vi "Test Instrument Remote API.vi"   [LabVIEW 2019]
uses:
  <vilib>/JKI/JKI SMO/SMO/Typedefs/SMOState --Enum.ctl
  c5a0c80c-7090-426d-a2a1-7f80a9253fe7.vi
  c5a0c80c-7090-426d-a2a1-7f80a9253fe7.vi/3f0cefdb-5cc5-4526-b0b8-38505ee8bd1c.vi
  c5a0c80c-7090-426d-a2a1-7f80a9253fe7.vi/3f0cefdb-5cc5-4526-b0b8-38505ee8bd1c.vi/fd19d2b7-c57e-488d-b648-4f9bde0d7289.vi
  c5a0c80c-7090-426d-a2a1-7f80a9253fe7.vi/3f0cefdb-5cc5-4526-b0b8-38505ee8bd1c.vi/0dd6771b-0bcd-4917-9756-116636ca7f0a.vi
  <vilib>/Utility/Data Type/Get Type Information.vi
  <vilib>/JDP Science/JSONtext/JSON text to Variant.vi
  <vilib>/addons/_JKI Toolkits/Caraya/classes/Assert/Assert Equal Value and Type_Variant.vi
  <vilib>/addons/_JKI Toolkits/Caraya/classes/Assert/Assert Not Error.vi
  <vilib>/JDP Science/JSONtext/LVClass Serializer/JSONtext LVClass Serializer.lvclass
  lvsrc/Framework/Instrument/Instrument.lvclass
  <vilib>/JKI/JKI SMO/SMO/SMO.lvclass
  <vilib>/addons/_JKI Toolkits/Caraya/classes/Assert/Assert.lvclass
  <vilib>/addons/_JKI Toolkits/Caraya/classes/Test/Test.lvclass
  lvsrc/Framework-Template/SMOs/Instrument.Framework-Template/Instrument.Framework-Template.lvclass
  C:/Users/patrick/Documents/GitHub/Instrument-Framework/lvsrc/Framework/Instrument Types/SCPI/Instrument.SCPI.lvclass
  C:/Users/patrick/Documents/GitHub/Instrument-Framework/lvsrc/Framework/Instrument/Instrument.lvclass
  C:/Program Files (x86)/National Instruments/LabVIEW 2019/vi.lib/JKI/JKI SMO/SMO/SMO.lvclass
types:
  T1 = typedef "SMO.lvclass/SMOState --Enum.ctl" = enum16{"unknown", "Created", "Started", "Stopped"}
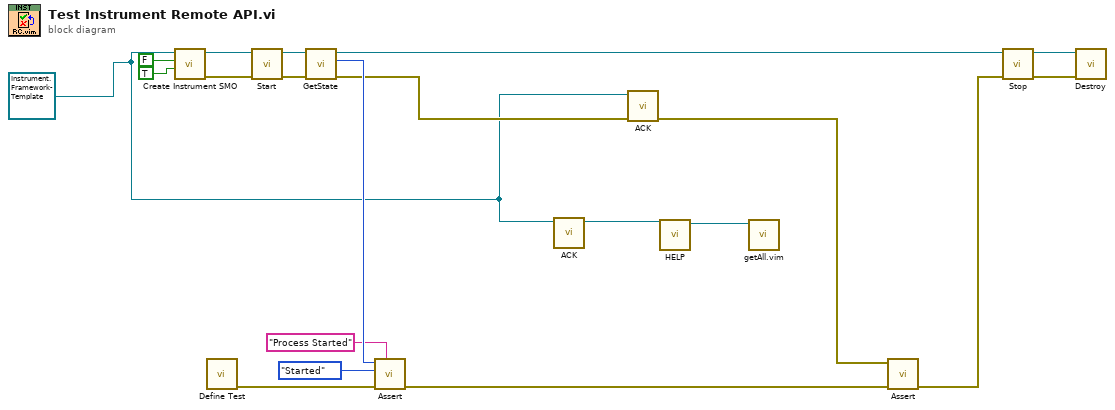
[diagram p0: block diagram]
diagram:
  w1 = refnum<class "Instrument.Framework-Template.lvclass"> refnum ("Instrument.Framework-Template.lvclass")
  n1 = call "Create Instrument SMO.vi"("Debug Mode? [F]"=TRUE, "Configuration Window? [T]"=FALSE, "Instrument in"=w1) -> ("error out"=w18:errorcluster, "Instrument in"=w19:refnum<class "Instrument.Framework-Template.lvclass">)  [unwired: 7 in]
  n2 = call <vilib>:"Define Test.vi"() -> ("error out"=w11:errorcluster)  [unwired: 10 in, 1 out]
  n3 = call <vilib>:"Start.vi"("error in (no error)"=w18, "SMO"=w19) -> ("error out"=w15:errorcluster, "SMO"=w14:refnum<class "Instrument.Framework-Template.lvclass">)  [unwired: 8 in]
  n4 = call <vilib>:"GetState.vi"("error in (no error)"=w15, "SMO"=w14) -> ("error out"=w4:errorcluster, "SMO State"=w13:T1, "SMO"=w5:refnum<class "Instrument.Framework-Template.lvclass">)  [unwired: 7 in]
  n5 = call-poly <vilib>:"Assert.vi"("Label"="Process Started", "error in (no error)"=w11, "Y"=SMOState_--Enum."Started" ("SMO State"), "X"=w13) -> ("error out"=w9:errorcluster)  [unwired: 6 in, 1 out]
  n6 = call "ACK.vi"("Instrument in"=w1) -> ("Instrument in"=w3:refnum<class "Instrument.Framework-Template.lvclass">)  [unwired: 8 in, 2 out]
  n7 = call "ACK.vi"("error in (no error)"=w4, "Instrument in"=w1) -> ("error out"=w8:errorcluster)  [unwired: 7 in, 2 out]
  n8 = call "HELP.vi"("Instrument in"=w3) -> ("Instrument in"=w2:refnum<class "Instrument.Framework-Template.lvclass">)  [unwired: 8 in, 2 out]
  n9 = call "getAll.vim"("Instrument in"=w2) -> ()  [unwired: 8 in, 3 out]
  n10 = call-poly <vilib>:"Assert.vi"("error in (no error)"=w9, "Not Error?"=w8) -> ("error out"=w7:errorcluster)  [unwired: 8 in, 1 out]
  n11 = call <vilib>:"Stop.vi"("error in (no error)"=w7, "SMO"=w5) -> ("error out"=w16:errorcluster, "SMO"=w17:refnum<class "Instrument.Framework-Template.lvclass">)  [unwired: 8 in]
  n12 = call <vilib>:"Destroy.vi"("error in (no error)"=w16, "SMO"=w17) -> ()  [unwired: 9 in, 1 out]
